vi "syd-PhasicFunctionv2.vi"() -> ()   [LabVIEW 2025]
uses:
  <vilib>/DAQmx/read.llb/DAQmx Read (Analog 1D Wfm NChan NSamp).vi
  <vilib>/DAQmx/create/channels.llb/DAQmx Create Channel (AI-Voltage-Basic).vi
  <vilib>/DAQmx/configure/timing.llb/DAQmx Timing (Sample Clock).vi
  <vilib>/DAQmx/miscellaneous.llb/DAQmx Fill In Error Info.vi
panel:
  out "Waveform Chart":waveform(dbl)[](graph)
  in  "error in":errorcluster
  out "data 2":waveform(dbl)[](graph) caption="data"
  in  "stop 2":bool caption="stop"
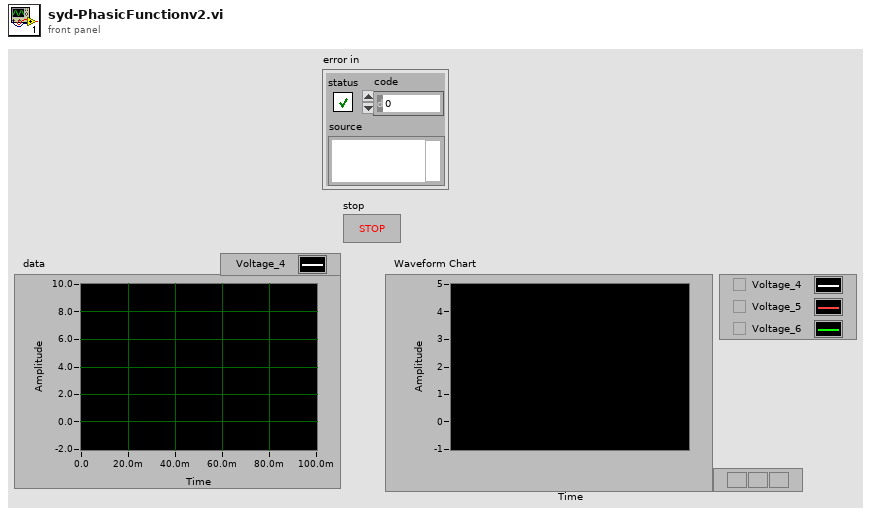
[diagram p1: front panel]
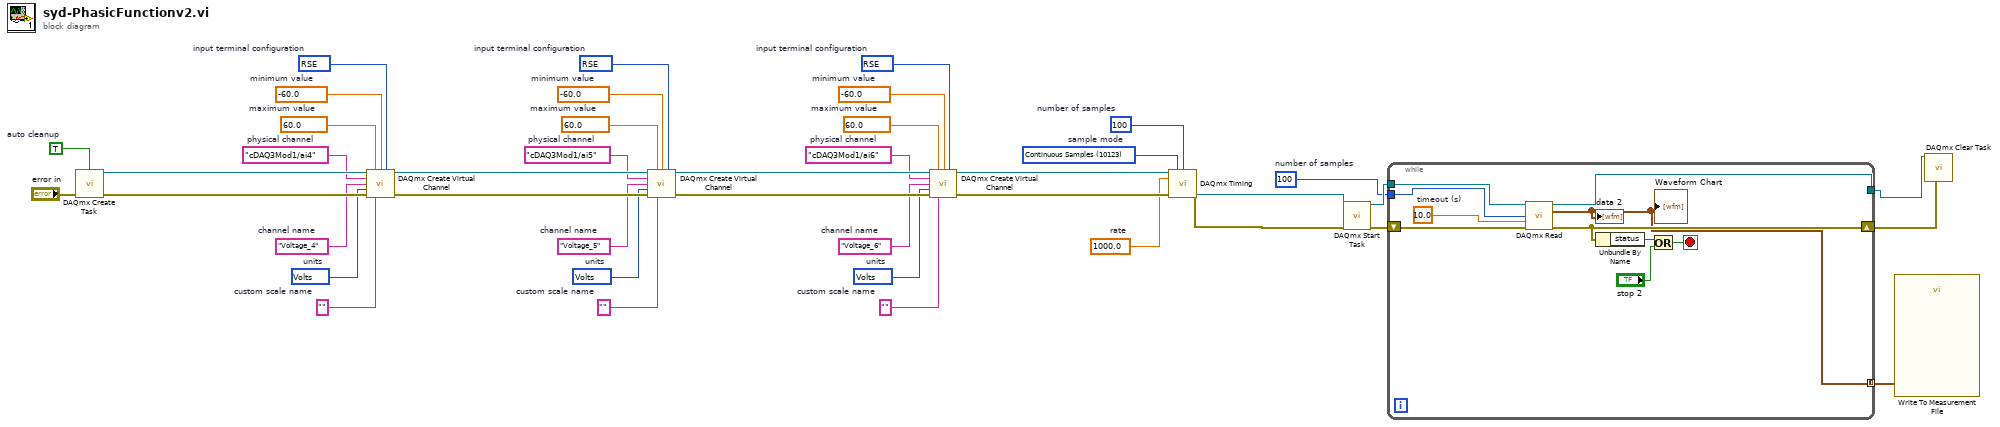
[diagram p0: block diagram]
diagram:
  w4 = 10123 items=["Finite Samples"=10178, "Continuous Samples"=10123, "Hardware Timed Single Point"=12522]  # sample mode
  w5 = 100  # number of samples
  w6 = 1000.0  # rate
  w8 = 10083 items=["default"=-1, "RSE"=10083, "NRSE"=10078, "Differential"=10106, "Pseudodifferential"=12529]  # input terminal configuration
  w9 = 10348 items=["Volts"=10348, "From Custom Scale"=10065]  # units
  w10 = "Voltage_6"  # channel name
  w12 = ""  # custom scale name
  w13 = -60.0  # minimum value
  w14 = 60.0  # maximum value
  w15 = "cDAQ3Mod1/ai6"  # physical channel
  w17 = 10083 items=["default"=-1, "RSE"=10083, "NRSE"=10078, "Differential"=10106, "Pseudodifferential"=12529]  # input terminal configuration
  w18 = 10348 items=["Volts"=10348, "From Custom Scale"=10065]  # units
  w19 = "Voltage_5"  # channel name
  w21 = ""  # custom scale name
  w22 = -60.0  # minimum value
  w23 = 60.0  # maximum value
  w24 = "cDAQ3Mod1/ai5"  # physical channel
  w26 = 10083 items=["default"=-1, "RSE"=10083, "NRSE"=10078, "Differential"=10106, "Pseudodifferential"=12529]  # input terminal configuration
  w27 = 10348 items=["Volts"=10348, "From Custom Scale"=10065]  # units
  w28 = "Voltage_4"  # channel name
  w30 = ""  # custom scale name
  w31 = -60.0  # minimum value
  w32 = 60.0  # maximum value
  w33 = "cDAQ3Mod1/ai4"  # physical channel
  w35 = TRUE  # auto cleanup
  w40 = 100  # number of samples
  n1 = call <vilib>:"DAQmx Create Task.vi"("auto cleanup"=w35, "error in"="error in") -> ("task out"=w34:refnum<k21>, "error out"=w36:errorcluster)  [unwired: 12 in]
  n2 = call-poly <vilib>:"DAQmx Create Virtual Channel.vi"("task in"=w34, "maximum value"=w32, "minimum value"=w31, "input terminal configuration"=w26, "physical channels"=w33, "name to assign"=w28, "units"=w27, "error in"=w36, "custom scale name"=w30) -> ("task out"=w25:refnum<k21>, "error out"=w29:errorcluster)  [unwired: 5 in]
  n3 = call-poly <vilib>:"DAQmx Create Virtual Channel.vi"("task in"=w25, "maximum value"=w23, "minimum value"=w22, "input terminal configuration"=w17, "physical channels"=w24, "name to assign"=w19, "units"=w18, "error in"=w29, "custom scale name"=w21) -> ("task out"=w16:refnum<k21>, "error out"=w20:errorcluster)  [unwired: 5 in]
  n4 = call-poly <vilib>:"DAQmx Create Virtual Channel.vi"("task in"=w16, "maximum value"=w14, "minimum value"=w13, "input terminal configuration"=w8, "physical channels"=w15, "name to assign"=w10, "units"=w9, "error in"=w20, "custom scale name"=w12) -> ("task out"=w7:refnum<k21>, "error out"=w11:errorcluster)  [unwired: 5 in]
  n5 = call-poly <vilib>:"DAQmx Timing.vi"("task/channels in"=w7, "sample mode"=w4, "samples per channel"=w5, "rate"=w6, "error in"=w11) -> ("task out"=w2:refnum<k21>, "error out"=w3:errorcluster)  [unwired: 9 in]
  n6 = call <vilib>:"DAQmx Start Task.vi"("task/channels in"=w2, "error in"=w3) -> ("task out"=w42:refnum<k21>, "error out"=w41:errorcluster)  [unwired: 12 in]
  n7 = while {
    tunnel: w42 -> [w52]
    tunnel: w40 -> [w49]
    tunnel: [w50] -> w38
    shift-right: [w47] -> w39
    shift-left: w41 -> [w51]
    tunnel: [w43] -> w1 mode=concatenating
    stop <- w46 stop-if-true
    w44 = 10.0  # timeout (s)
    n8 = call-poly <vilib>:"DAQmx Read.vi"("task/channels in"=w52, "number of samples per channel"=w49, "timeout"=w44, "error in"=w51) -> ("task out"=w50:refnum<k21>, "data"=w43:waveform(dbl)[], "error out"=w47:errorcluster)  [unwired: 9 in]
    "data 2" <- w43
    "Waveform Chart" <- w43
    n9 = Unbundle By Name(w47) -> ("status"=w48:bool)
    n10 = Or(x=w48, y="stop 2") -> (x .or. y?=w46:bool)
  }
  n11 = call "Write To Measurement File"("Signals"=w1) -> ()  [unwired: 16 in, 3 out]
  n12 = call <vilib>:"DAQmx Clear Task.vi"("task in"=w38, "error in"=w39) -> ()  [unwired: 13 in, 1 out]
